vi "Pack for gRPC.vi"(8 "error in":errorcluster, 9 "configuration / results":enum16{"Configuration", "Results"}(ring), 10 "data value":variant, 11 "measurement customizations in":refnum<class "Measurement Plugin.lvclass">) -> (0 "error out":errorcluster, 2 "any":T1, 3 "measurement customizations out":refnum<class "Measurement Plugin.lvclass">)   [LabVIEW 2021, in "PSRR_PMIC.lvlib" / "Measurement Plugin.lvclass"]
uses:
  Measurement Plugin.lvclass
  <vilib>/gRPC/LabVIEW gRPC Library/Shared/Any.ctl
  C:/Program Files/National Instruments/LabVIEW 2021/vi.lib/Plug-In SDKs/Measurements/Measurement Plugin Service/Measurement Plugin Service.lvclass
  Measurement Configuration.ctl
  Measurement Results.ctl
  2eca732d-dbaa-43bf-a7dd-ede2da65bc1b.vi
  a6012965-5700-4384-8228-972e71b6560c.vi
  <vilib>/gRPC/LabVIEW gRPC Library/Server API/Translate Protobuf Error.vi
  <vilib>/AdvancedString/1D String Array to Delimited String.vi
  <vilib>/gRPC/LabVIEW gRPC Library/Server API/Server/Get Server DLL Path.vi
  Measurement Plugin.lvclass/Measurement Plugin.ctl
  PSRR_PMIC.lvlib
  <vilib>/Plug-In SDKs/Measurements/Measurement Plugin Service/Measurement Plugin Service.lvclass
  <vilib>/gRPC/LabVIEW gRPC Library/grpc-lvsupport-release.lvlib
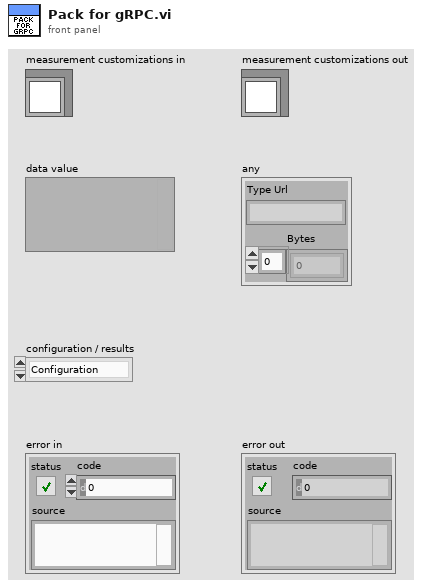
[diagram p1: front panel]
types:
  T1 = typedef "grpc-lvsupport-release.lvlib/Any.ctl" = cluster{"Type Url":string, "Bytes":u8[]}
  T2 = typedef "grpc-lvsupport-release.lvlib/grpcId.ctl" = u64
  T3 = typedef "PSRR_PMIC.lvlib/Measurement Configuration.ctl" = cluster{"DUT setup time":dbl, "Source resource name":string, "Source current limit":dbl, "Source voltage level":dbl, "Load resource name":string, "Load voltage limit range":dbl, "Load current level":dbl, "Fgen resource name":string, "Fgen channel name":string, "Fgen pk-pk amplitude":dbl, "Fgen load impedance":dbl, "Fgen start frequency":dbl, "Fgen stop frequency":dbl, "Fgen frequency sweep points/points per decade":i32, "Fgen sweep type":string, "Fgen standard Waveform":enum32{"Sine", "Square", "Triangle", "Ramp Up", "Ramp Down", "DC", "Noise"}, "Scope resource name":string, "Scope input channel name":string, "Scope output channel name":string, "Scope probe attenuation":dbl, "Scope samples per cycle":i32, "Scope cycles to average":i32}
  T4 = typedef "PSRR_PMIC.lvlib/Measurement Results.ctl" = cluster{"Frequency sweep points":dbl[], "PSRR":dbl[]}
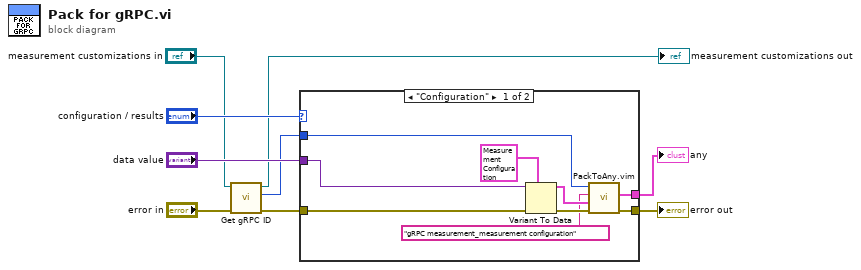
[diagram p0: block diagram]
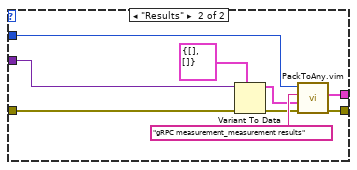
[diagram p2: hidden frame]
diagram:
  n1 = call <vilib>:"Get gRPC ID.vi"("error in"="error in", "measurement plugin service in"="measurement customizations in") -> ("error out"=w4:errorcluster, "gRPC ID"=w1:T2, "measurement plugin service out"=→"measurement customizations out":refnum<class "Measurement Plugin.lvclass">)  [unwired: 7 in]
  n2 = case shown="\"Configuration\"" "configuration / results" {
    tunnel: w4 -> [w18 w27]
    tunnel: "data value" -> [w17 w26]
    tunnel: w1 -> [w14 w22]
    tunnel: [w16 w24] -> w8
    tunnel: [w15 w23] -> w7
    frame "Configuration" {
      n3 = Variant To Data(error in=w18, type=T3 {"DUT setup time"=1.0, "Source resource name"="", "Source current limit"=0.15, "Source voltage level"=10.0, "Load resource name"="", "Load voltage limit range"=6.0, "Load current level"=0.025, "Fgen resource name"="", "Fgen channel name"="", "Fgen pk-pk amplitude"=1.0, "Fgen load impedance"=10000.0, "Fgen start frequency"=10.0, "Fgen stop frequency"=10000000.0, "Fgen frequency sweep points/points per decade"=10, "Fgen sweep type"="Logarithmic", "Fgen standard Waveform"=enum."Sine", "Scope resource name"="", "Scope input channel name"="", "Scope output channel name"="", "Scope probe attenuation"=1.0, "Scope samples per cycle"=1000, "Scope cycles to average"=4} ("measurement configuration"), Variant=w17) -> (data=w13:T3, error out=w12:errorcluster)
      n4 = call "PackToAny.vim"("error in"=w12, "Data To Pack"=w13, "Message Type"="gRPC measurement_measurement configuration", "gRPCid in"=w14) -> ("error out"=w16:errorcluster, "Any"=w15:T1)  [unwired: 5 in, 1 out]
    }
    frame "Results" {
      n5 = Variant To Data(error in=w27, type=T4 {"Frequency sweep points"=[], "PSRR"=[]} ("Measurement Results"), Variant=w26) -> (data=w20:T4, error out=w19:errorcluster)
      n6 = call "PackToAny.vim"("error in"=w19, "Data To Pack"=w20, "Message Type"="gRPC measurement_measurement results", "gRPCid in"=w22) -> ("error out"=w24:errorcluster, "Any"=w23:T1)  [unwired: 5 in, 1 out]
    }
  }
  "error out" <- w8
  "any" <- w7
